vi "LED.vi"(2 "Speed":u8, 3 "IP":string, 4 "Length":u8, 5 "Brightness":u8, 6 "Color":u8, 7 "Direction":u8) -> ()   [LabVIEW 2026]
panel:
  out "Port":dbl
  in  "Send":bool
  # "LED Light Strip Control"
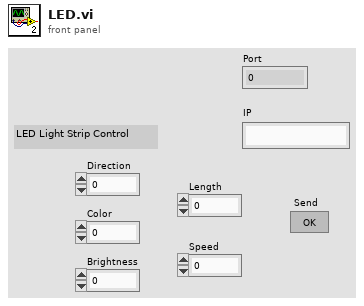
[diagram p1: front panel]
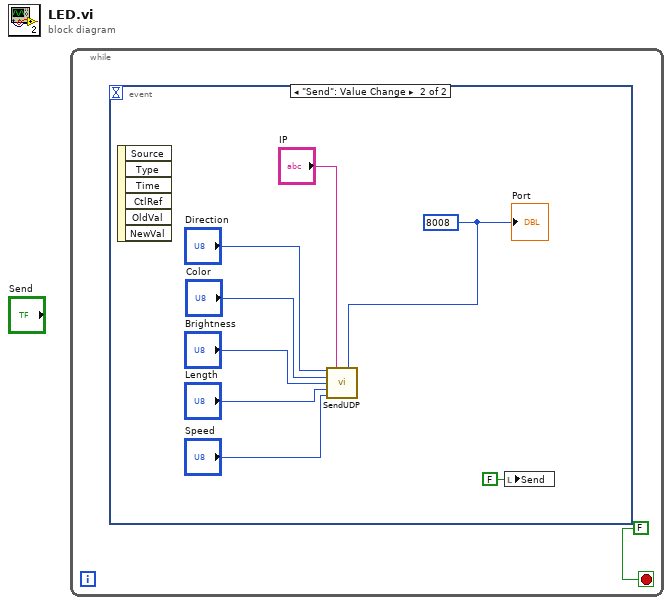
[diagram p0: block diagram]
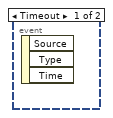
[diagram p2: hidden frame]
diagram:
  n1 = while {
    stop <- FALSE stop-if-true
    n2 = event shown="[1] \"Send\": Value Change" {
      selector: _ -> [_ _]
      dyn-events: _ -> [_ _]
      timeout: _ -> [_ _]
      event Timeout {
        n3 = event-data() -> ()  [unwired: 1 in, 3 out]
      }
      event "Send": Value Change {
        w8 = 8008
        n4 = event-data() -> ()  [unwired: 1 in, 6 out]
        n5 = call "SendUDP.vi"("Arg3"="Direction", "IP"="IP", "Port"=w8, "Arg4"="Color", "Arg5"="Brightness", "Arg6"="Length", "Arg7"="Speed") -> ()  [unwired: 9 in]
        n6 = local write "Send"(FALSE ("Send")) -> ()
        "Port" <- w8
      }
    }
  }
